vi "Update.vi"(4 "Headphone Block 2":dbl[][](array[numeric]), 6 "Headphone Block 1":dbl[][](array[numeric]), 8 "error in (no error)":errorcluster, 9 "Audio Block 2":dbl[][](array[numeric]), 10 "Audio Block 1":dbl[][](array[numeric]), 11 "Mixer in":refnum<class "Mixer.lvclass">) -> (0 "error out":errorcluster, 1 "Headphones Audio Block Out":dbl[][](array[numeric]), 2 "Master Audio Block Out":dbl[][](array[numeric]), 3 "Mixer out":refnum<class "Mixer.lvclass">)   [LabVIEW 2019, in "Mixer.lvclass"]
uses:
  Mixer.lvclass
  Mixer.lvclass/Mixer.ctl
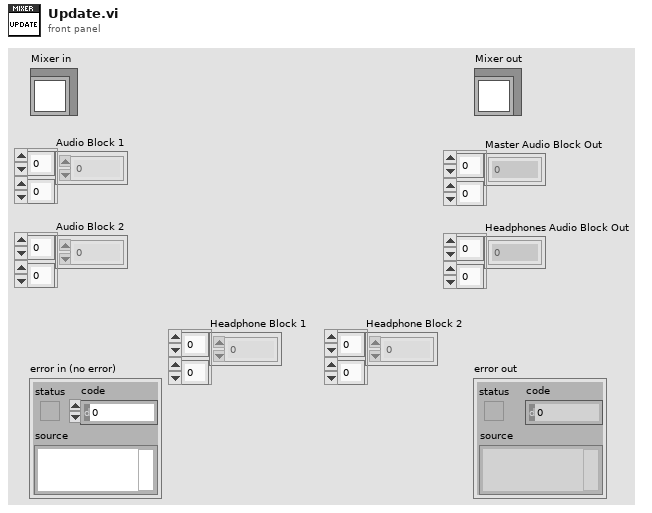
[diagram p1: front panel]
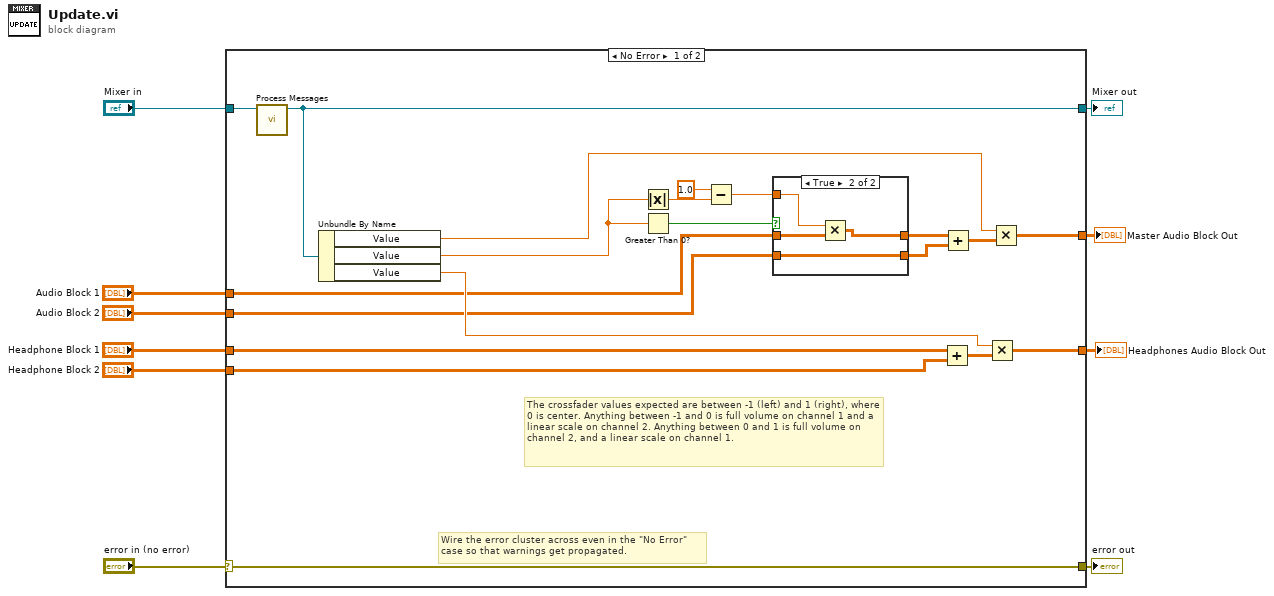
[diagram p0: block diagram]
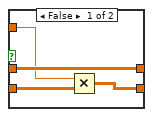
[diagram p2: hidden frame]
diagram:
  n1 = case shown="No Error" "error in (no error)" {
    selector: "error in (no error)" -> [w30 w41]
    tunnel: [w30 w41] -> w9
    tunnel: [w14 w40] -> w7
    tunnel: "Mixer in" -> [w29 w40]
    tunnel: "Audio Block 1" -> [w15 w39]
    tunnel: "Audio Block 2" -> [w13 _]
    tunnel: [w19 w39] -> w4
    tunnel: [w16 w39] -> w3
    tunnel: "Headphone Block 1" -> [w12 _]
    tunnel: "Headphone Block 2" -> [w11 _]
    frame No Error {
      # "The crossfader values expected are between -1 (left) and 1 (right), where 0 is center. Anything between -1 and 0 is full volume on channel 1 and a linear scale on channel 2. Anything between 0 and 1 is full volume on channel 2, and a linear scale on channel 1."
      # "Wire the error cluster across even in the \"No Error\"\ncase so that warnings get propagated."
      n2 = call "Process Messages.vi"("Mixer in"=w29) -> ("Mixer out"=w14:refnum<class "Mixer.lvclass">)  [unwired: 9 in, 1 out]
      n3 = Unbundle By Name(w14) -> ("Value"=w20:dbl, "Value"=w27:dbl, "Value"=w17:dbl)
      n4 = Absolute Value(x=w27) -> (abs(x)=w25:dbl)
      n5 = Greater Than 0?(x=w27) -> (x > 0?=w28:bool)
      n6 = Subtract(x=1.0, y=w25) -> (x-y=w24:dbl)
      n7 = case shown="True" w28 {
        tunnel: w15 -> [w32 w37]
        tunnel: w13 -> [w34 w38]
        tunnel: w24 -> [w31 w36]
        tunnel: [w33 w38] -> w22
        tunnel: [w32 w35] -> w23
        frame False {
          n8 = Multiply(x=w31, y=w34) -> (x*y=w33:dbl[][])
        }
        frame True {
          n9 = Multiply(x=w36, y=w37) -> (x*y=w35:dbl[][])
        }
      }
      n10 = Add(x=w12, y=w11) -> (x+y=w18:dbl[][])
      n11 = Add(x=w23, y=w22) -> (x+y=w21:dbl[][])
      n12 = Multiply(x=w17, y=w18) -> (x*y=w16:dbl[][])
      n13 = Multiply(x=w20, y=w21) -> (x*y=w19:dbl[][])
    }
    frame Error {
    }
  }
  "error out" <- w9
  "Mixer out" <- w7
  "Master Audio Block Out" <- w4
  "Headphones Audio Block Out" <- w3
